vi "Write Connected_.vi"(8 "error in (no error)":errorcluster, 10 "Connected?":bool, 11 "FSV-40N in":refnum<class "FSV-40N.lvclass">) -> (0 "error out":errorcluster, 3 "FSV-40N out":refnum<class "FSV-40N.lvclass">)   [LabVIEW 2023, in "Spectrum Analyzer.lvlib" / "FSV-40N.lvclass"]
uses:
  FSV-40N.lvclass
  FSV-40N.lvclass/FSV-40N.ctl
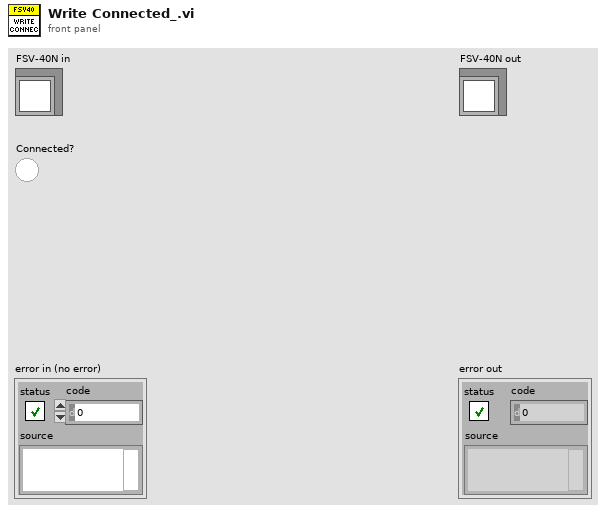
[diagram p1: front panel]
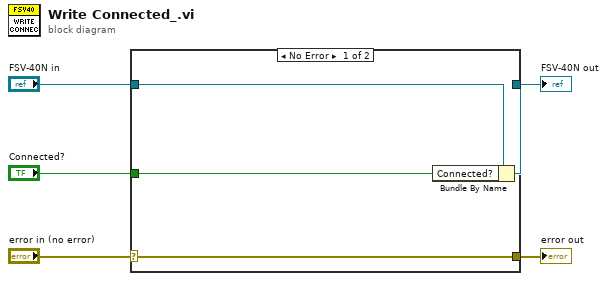
[diagram p0: block diagram]
diagram:
  n1 = case shown="No Error" "error in (no error)" {
    selector: "error in (no error)" -> [w9 w10]
    tunnel: [w9 w10] -> w4
    tunnel: [w7 w11] -> w2
    tunnel: "FSV-40N in" -> [w8 w11]
    tunnel: "Connected?" -> [w6 _]
    frame No Error {
      n2 = Bundle By Name(cluster=w8, "Connected?"=w6) -> (w7:refnum<class "FSV-40N.lvclass">)
    }
    frame Error {
    }
  }
  "error out" <- w4
  "FSV-40N out" <- w2
